vi "MQTT Reason TEXT.vi"(5 "Message Type":T1, 7 "Reason Code":u8) -> (8 "Reason Text":string)   [LabVIEW 2019, in "KoRE-MQTT.lvlib"]
doc: "Copyright (c) 2025 KoRElibs.com\nSPDX-License-Identifier: EUPL-1.2\n\nThis VI is licensed under the European Union Public License (EUPL) Version 1.2. You may use this VI unmodified in proprietary works. If you distribute a modified version of this file, the modified file must be released under the EUPL-1.2. Full license: https://joinup.ec.europa.eu/asset/eupl/eupl/1.2/"
uses:
  KoRE-MQTT.lvlib
  TypeDefs/MQTT Packet - Type.ctl
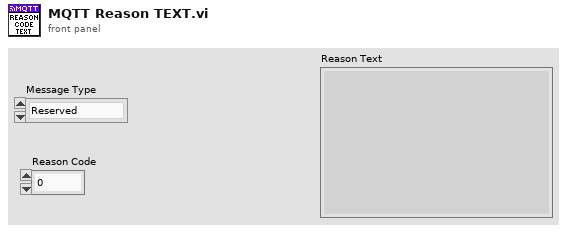
[diagram p1: front panel]
types:
  T1 = typedef "KoRE-MQTT.lvlib/MQTT Packet - Type.ctl" = enum32{"Reserved", "CONNECT", "CONNACK", "PUBLISH", "PUBACK", "PUBREC", "PUBREL", "PUBCOMP", "SUBSCRIBE", "SUBACK", "UNSUBSCRIBE", "UNSUBACK", "PINGREQ", "PINGRESP", "DISCONNECT", "AUTH"}
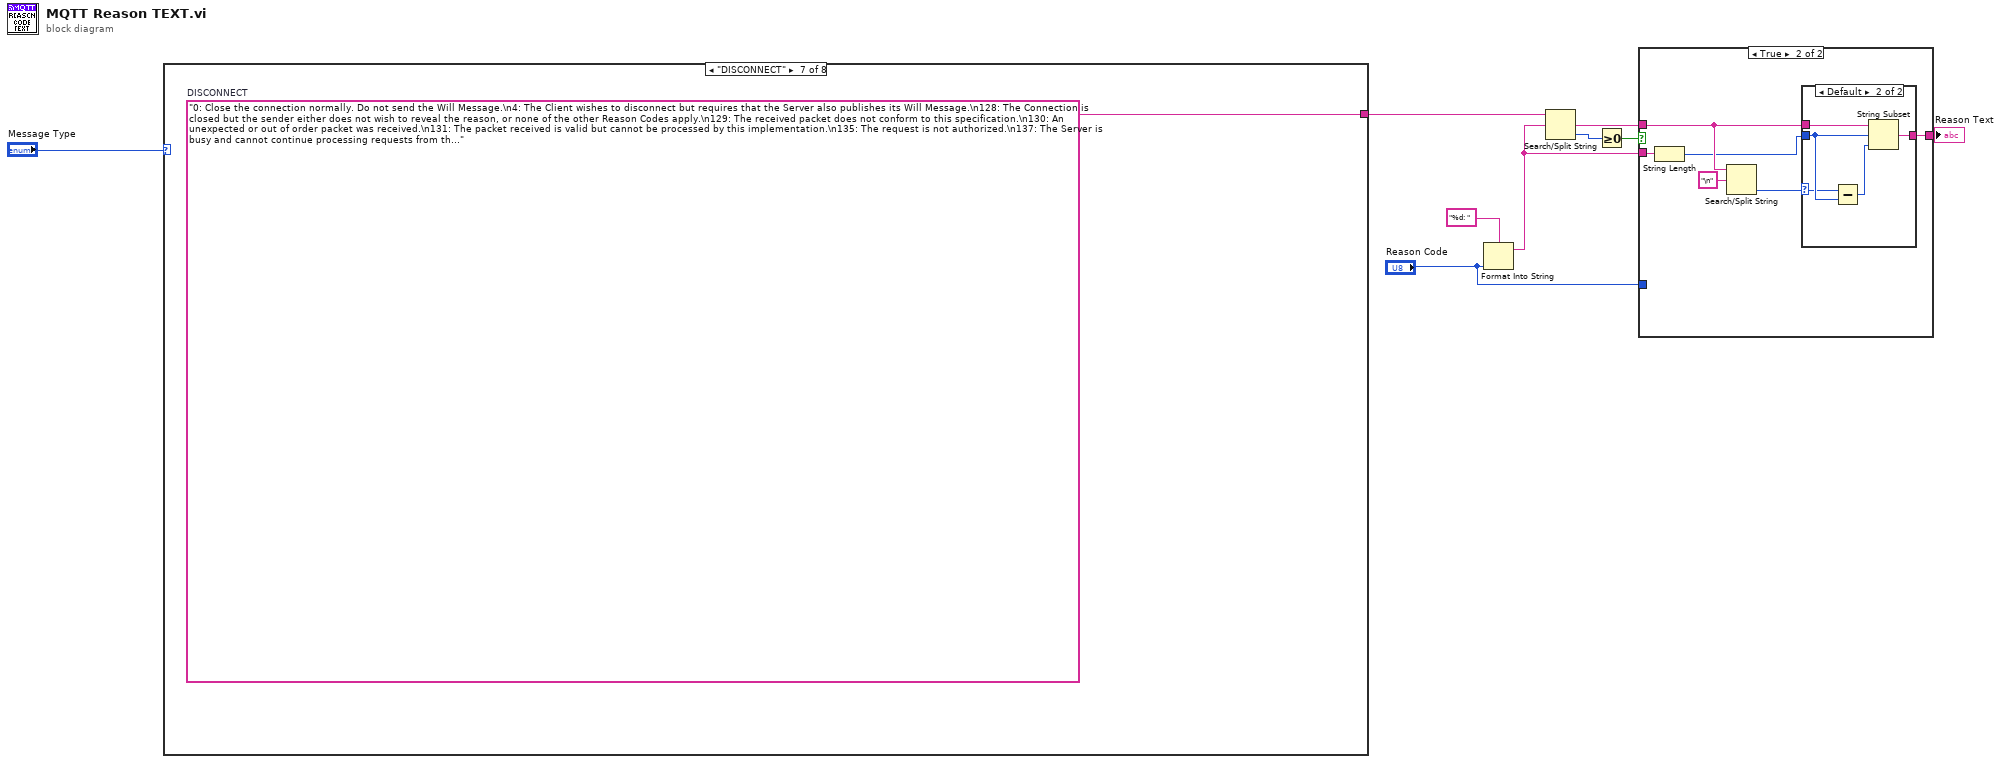
[diagram p0: block diagram]
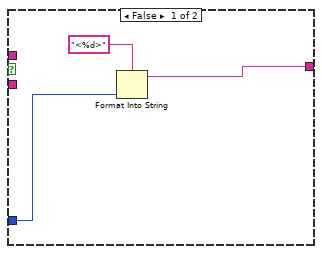
[diagram p2: hidden frame]
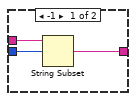
[diagram p3: hidden frame]
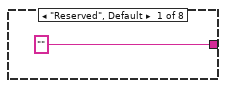
[diagram p4: hidden frame]
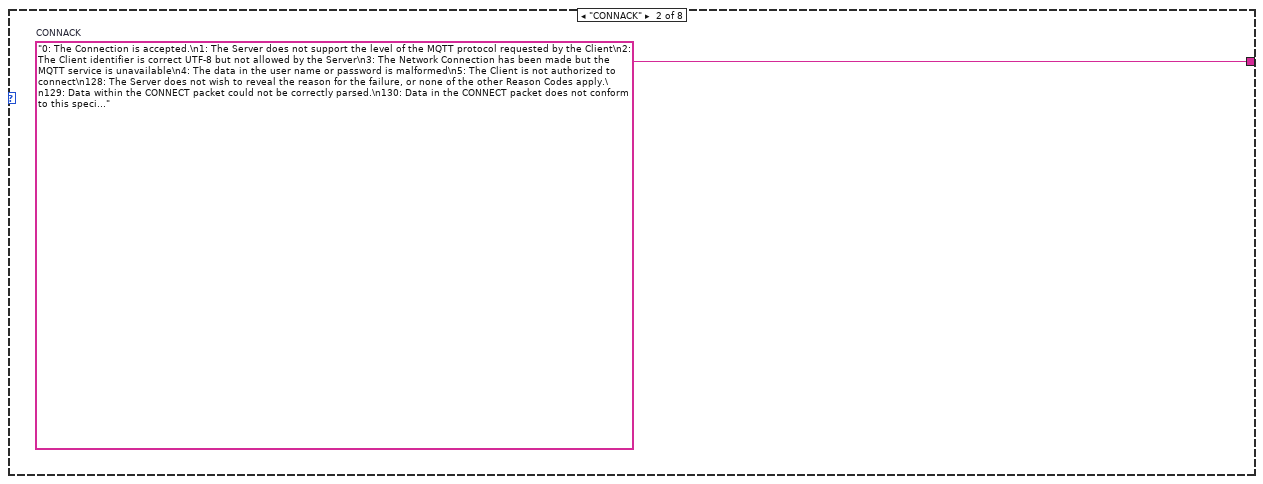
[diagram p5: hidden frame]
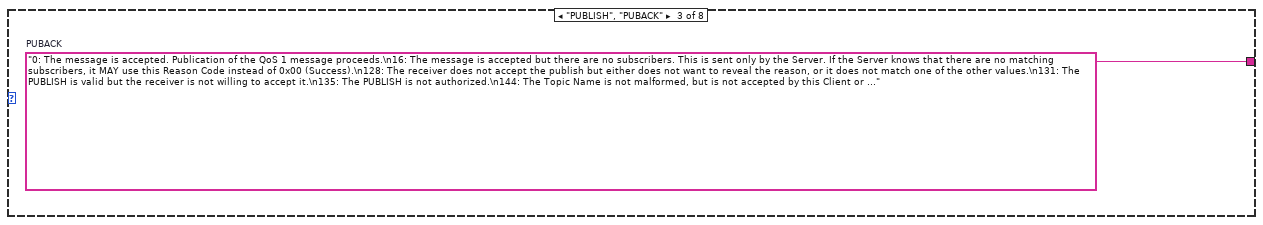
[diagram p6: hidden frame]
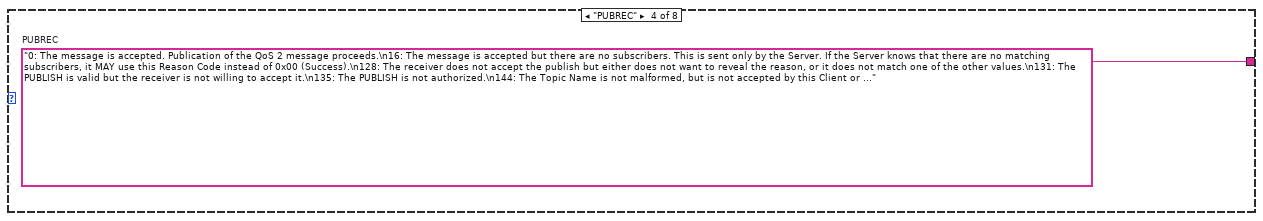
[diagram p7: hidden frame]
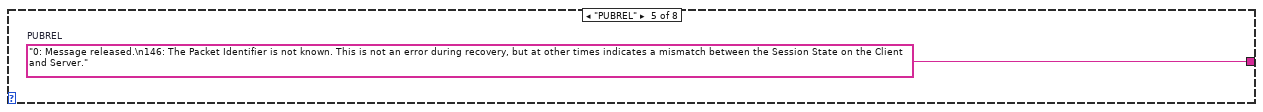
[diagram p8: hidden frame]
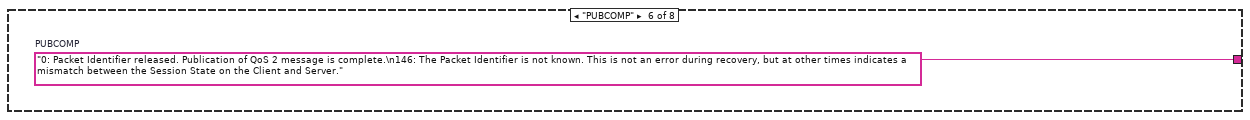
[diagram p9: hidden frame]
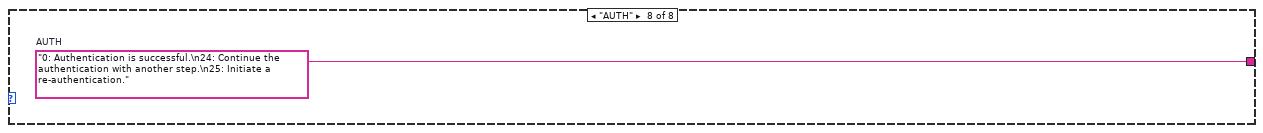
[diagram p10: hidden frame]
diagram:
  n1 = case shown="\"DISCONNECT\"" "Message Type" {
    tunnel: ["" ("AUTH") w11 w12 w13 w14 w15 w16 w17] -> w8
    frame "Reserved", Default {
    }
    frame "CONNACK" {
      w11 = "0: The Connection is accepted.\n1: The Server does not support the level of the MQTT protocol requested by the Client\n2: The Client identifier is correct UTF-8 but not allowed by the Server\n3: The Network Connection has been made but the MQTT service is unavailable\n4: The data in the user name or password is malformed\n5: The Client is not authorized to connect\n128: The Server does not wish to reveal the reason for the failure, or none of the other Reason Codes apply.\n129: Data within the CONNECT packet could not be correctly parsed.\n130: Data in the CONNECT packet does not conform to this specification.\n131: The CONNECT is valid but is not accepted by this Server.\n132: The Server does not support the version of the MQTT protocol requested by the Client.\n133: The Client Identifier is a valid string but is not allowed by the Server.\n134: The Server does not accept the User Name or Password specified by the Client.\n135: The Client is not authorized to connect.\n136: The MQTT Server is not available.\n137: The Server is busy. Try again later.\n138: This Client has been banned by administrative action. Contact the server administrator.\n140: The authentication method is not supported or does not match the authentication method currently in use.\n144: The Will Topic Name is not malformed, but is not accepted by this Server.\n149: The CONNECT packet exceeded the maximum permissible size.\n151: An implementation or administrative imposed limit has been exceeded.\n153: The Will Payload does not match the specified Payload Format Indicator.\n154: The Server does not support retained messages, and Will Retain was set to 1.\n155: The Server does not support the QoS set in Will QoS.\n156: The Client should temporarily use another server.\n157: The Client should permanently use another server.\n159: The connection rate limit has been exceeded."  # CONNACK
    }
    frame "PUBLISH", "PUBACK" {
      w12 = "0: The message is accepted. Publication of the QoS 1 message proceeds.\n16: The message is accepted but there are no subscribers. This is sent only by the Server. If the Server knows that there are no matching subscribers, it MAY use this Reason Code instead of 0x00 (Success).\n128: The receiver does not accept the publish but either does not want to reveal the reason, or it does not match one of the other values.\n131: The PUBLISH is valid but the receiver is not willing to accept it.\n135: The PUBLISH is not authorized.\n144: The Topic Name is not malformed, but is not accepted by this Client or Server.\n145: The Packet Identifier is already in use. This might indicate a mismatch in the Session State between the Client and Server.\n151: An implementation or administrative imposed limit has been exceeded.\n153: The payload format does not match the specified Payload Format Indicator."  # PUBACK
    }
    frame "PUBREC" {
      w13 = "0: The message is accepted. Publication of the QoS 2 message proceeds.\n16: The message is accepted but there are no subscribers. This is sent only by the Server. If the Server knows that there are no matching subscribers, it MAY use this Reason Code instead of 0x00 (Success).\n128: The receiver does not accept the publish but either does not want to reveal the reason, or it does not match one of the other values.\n131: The PUBLISH is valid but the receiver is not willing to accept it.\n135: The PUBLISH is not authorized.\n144: The Topic Name is not malformed, but is not accepted by this Client or Server.\n145: The Packet Identifier is already in use. This might indicate a mismatch in the Session State between the Client and Server.\n151: An implementation or administrative imposed limit has been exceeded.\n153: The payload format does not match the one specified in the Payload Format Indicator."  # PUBREC
    }
    frame "PUBREL" {
      w14 = "0: Message released.\n146: The Packet Identifier is not known. This is not an error during recovery, but at other times indicates a mismatch between the Session State on the Client and Server."  # PUBREL
    }
    frame "PUBCOMP" {
      w15 = "0: Packet Identifier released. Publication of QoS 2 message is complete.\n146: The Packet Identifier is not known. This is not an error during recovery, but at other times indicates a mismatch between the Session State on the Client and Server."  # PUBCOMP
    }
    frame "DISCONNECT" {
      w16 = "0: Close the connection normally. Do not send the Will Message.\n4: The Client wishes to disconnect but requires that the Server also publishes its Will Message.\n128: The Connection is closed but the sender either does not wish to reveal the reason, or none of the other Reason Codes apply.\n129: The received packet does not conform to this specification.\n130: An unexpected or out of order packet was received.\n131: The packet received is valid but cannot be processed by this implementation.\n135: The request is not authorized.\n137: The Server is busy and cannot continue processing requests from this Client.\n139: The Server is shutting down.\n141: The Connection is closed because no packet has been received for 1.5 times the Keepalive time.\n142: Another Connection using the same ClientID has connected causing this Connection to be closed.\n143: The Topic Filter is correctly formed, but is not accepted by this Server.\n144: The Topic Name is correctly formed, but is not accepted by this Client or Server.\n147: The Client or Server has received more than Receive Maximum publication for which it has not sent PUBACK or PUBCOMP.\n148: The Client or Server has received a PUBLISH packet containing a Topic Alias which is greater than the Maximum Topic Alias it sent in the CONNECT or CONNACK packet.\n149: The packet size is greater than Maximum Packet Size for this Client or Server.\n150: The received data rate is too high.\n151: An implementation or administrative imposed limit has been exceeded.\n152: The Connection is closed due to an administrative action.\n153: The payload format does not match the one specified by the Payload Format Indicator.\n154: The Server does not support retained messages.\n155: The Client specified a QoS greater than the QoS specified in a Maximum QoS in the CONNACK.\n156: The Client should temporarily change its Server.\n157: The Server is moved and the Client should permanently change its server location.\n158: The Server does not support Shared Subscriptions.\n159: This connection is closed because the connection rate is too high.\n160: The maximum connection time authorized for this connection has been exceeded.\n161: The Server does not support Subscription Identifiers; the subscription is not accepted.\n162: The Server does not support Wildcard Subscriptions; the subscription is not accepted.\n255: The Server closed the connection for unknown reasons. The protocol version does not support DISCONNECT reason code."  # DISCONNECT
    }
    frame "AUTH" {
      w17 = "0: Authentication is successful.\n24: Continue the authentication with another step.\n25: Initiate a re-authentication."  # AUTH
    }
  }
  n2 = Format Into String(format string="%d: ", "Reason Code") -> (resulting string=w1:string)  [unwired: 2 in, 1 out]
  n3 = Search/Split String(string=w8, search string/char (-)=w1) -> (match + rest of string=w2:string, offset of match=w3:i32)  [unwired: 1 in, 1 out]
  n4 = Greater Or Equal To 0?(x=w3) -> (x >= 0?=w6:bool)
  n5 = case shown="True" w6 {
    tunnel: w2 -> [_ w26]
    tunnel: [w18 w24] -> w5
    tunnel: "Reason Code" -> [w19 _]
    tunnel: w1 -> [_ w23]
    frame False {
      n6 = Format Into String(format string="<%d>", w19) -> (resulting string=w18:string)  [unwired: 2 in, 1 out]
    }
    frame True {
      n7 = String Length(string=w23) -> (length=w21:i32)
      n8 = Search/Split String(string=w26, search string/char (-)="\n") -> (offset of match=w22:i32)  [unwired: 1 in, 2 out]
      n9 = case shown="Default" w22 {
        selector: w22 -> [_ w30]
        tunnel: w26 -> [w29 w34]
        tunnel: [w27 w33] -> w24
        tunnel: w21 -> [w28 w31]
        frame -1 {
          n10 = String Subset(string=w29, offset (0)=w28) -> (substring=w27:string)  [unwired: 1 in]
        }
        frame Default {
          n11 = Subtract(x=w30, y=w31) -> (x-y=w32:i32)
          n12 = String Subset(string=w34, offset (0)=w31, length (rest)=w32) -> (substring=w33:string)
        }
      }
    }
  }
  "Reason Text" <- w5
